vi "lvmcp_propitemset.vi"() -> ()   [LabVIEW 2015]
panel:
  out "error out":errorcluster
  in  "name":string
  in  "item":refnum<vi>
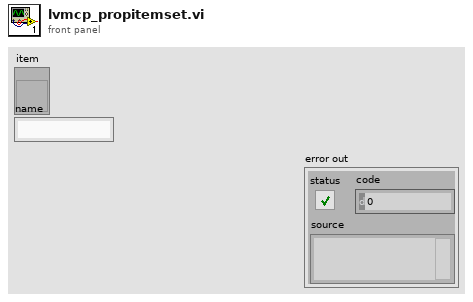
[diagram p1: front panel]
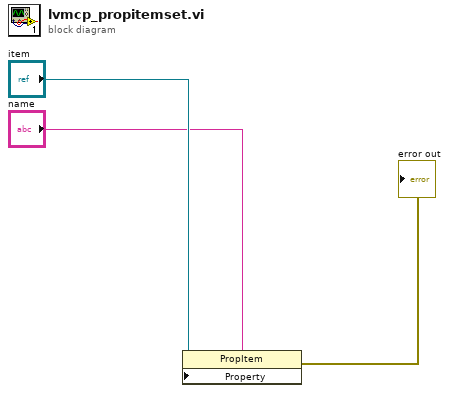
[diagram p0: block diagram]
diagram:
  n1 = property class="PropItem"(reference="item", "Property"="name") -> (error out=→"error out":errorcluster)  [unwired: 1 in, 1 out]
